vi "PhotonTrackedTarget_Pack.vi"(11 "TrackedTarget":T1={"Yaw"=0.0, "Pitch"=0.0, "Area"=0.0, "Skew"=0.0, "MinAreaRectCorners"=[], "BestCameraToTarget"={"TRANSLATION3D"={"X"=0.0, "Y"=0.0, "Z"=0.0}, "ROTATION3D"={"Q_quaternion"={"R"=1.0, "V"=[0.0, 0.0, 0.0]}}, "XF"=FALSE}, "FiducialId"=0, "AltCameraToTarget"={"TRANSLATION3D"={"X"=0.0, "Y"=0.0, "Z"=0.0}, "ROTATION3D"={"Q_quaternion"={"R"=1.0, "V"=[0.0, 0.0, 0.0]}}, "XF"=FALSE}, "PoseAmbiguity"=0.0, "DetectedCorners"=[], "ObjDetectId"=0, "ObjDetectConf"=0.0} {"AltCameraToTarget"."TRANSLATION3D"."Z" format="%14.3f"; "AltCameraToTarget"."TRANSLATION3D"."Y" format="%14.3f"; "AltCameraToTarget"."TRANSLATION3D"."X" format="%14.3f"; "BestCameraToTarget"."TRANSLATION3D"."Z" format="%14.3f"; "BestCameraToTarget"."TRANSLATION3D"."Y" format="%14.3f"; "BestCameraToTarget"."TRANSLATION3D"."X" format="%14.3f"}) -> (3 "RawData Out":u8[](array[numeric]))   [LabVIEW 2019, in "PhotonVisionLib.lvlib"]
doc: "Encode a TrackedTarget cluster into an array of bytes.\n\nInputs:\n - TrackedTarget -- TrackedTarget cluster.\n\nOutputs:\n - RawDataOut -- Byte array containing the encoded data."
uses:
  PhotonVisionLib.lvlib
  TypeDef/PhotonTrackedTargetType.ctl
  TypeDef/TargetCornerType.ctl
  <vilib>/Rock Robotics/WPI/ThirdParty/JAS_Junk/TrajLib/TypeDef/TRANSFORM3D.ctl
  <vilib>/Rock Robotics/WPI/ThirdParty/JAS_Junk/TrajLib/TypeDef/TRANSLATION3D.ctl
  <vilib>/Rock Robotics/WPI/ThirdParty/JAS_Junk/TrajLib/TypeDef/ROTATION3D.ctl
  <vilib>/Rock Robotics/WPI/ThirdParty/JAS_Junk/TrajLib/TypeDef/QUATERNION.ctl
  <vilib>/Rock Robotics/WPI/ThirdParty/JAS_Junk/TrajLib/VI/Transform3d_GetRotation3d.vi
  <vilib>/Rock Robotics/WPI/ThirdParty/JAS_Junk/TrajLib/VI/Transform3d_GetTranslation3d.vi
  <vilib>/Rock Robotics/WPI/ThirdParty/JAS_Junk/TrajLib/VI/Translation3d_ToTranslation2d.vi
  <vilib>/Rock Robotics/WPI/ThirdParty/JAS_Junk/TrajLib/VI/Rotation3d_ToRotation2d.vi
  <vilib>/Rock Robotics/WPI/ThirdParty/JAS_Junk/TrajLib/Transform2d_Create_TransRot.vi
  <vilib>/Rock Robotics/WPI/ThirdParty/JAS_Junk/TrajLib/VI/Transform3d_GetXYZ.vi
  <vilib>/Rock Robotics/WPI/ThirdParty/JAS_Junk/TrajLib/VI/Rotation3d_GetQuaterion.vi
  <vilib>/Rock Robotics/WPI/ThirdParty/JAS_Junk/TrajLib/VI/Quaternion_Get_All.vi
  Packet_encode_ByteI8.vi
  TargetCorner_GetAll.vi
  <vilib>/Rock Robotics/WPI/ThirdParty/JAS_Junk/TrajLib/Translation2d_Create.vi
  <vilib>/Rock Robotics/WPI/ThirdParty/JAS_Junk/TrajLib/Rotation2d_CreateAngle.vi
  <vilib>/Rock Robotics/WPI/ThirdParty/JAS_Junk/TrajLib/VI/Rotation3d_GetXYZ.vi
  <vilib>/Rock Robotics/WPI/ThirdParty/JAS_Junk/TrajLib/VI/Translation3d_GetXYZ.vi
  <vilib>/Rock Robotics/WPI/ThirdParty/JAS_Junk/TrajLib/Trajectory_Library.lvlib
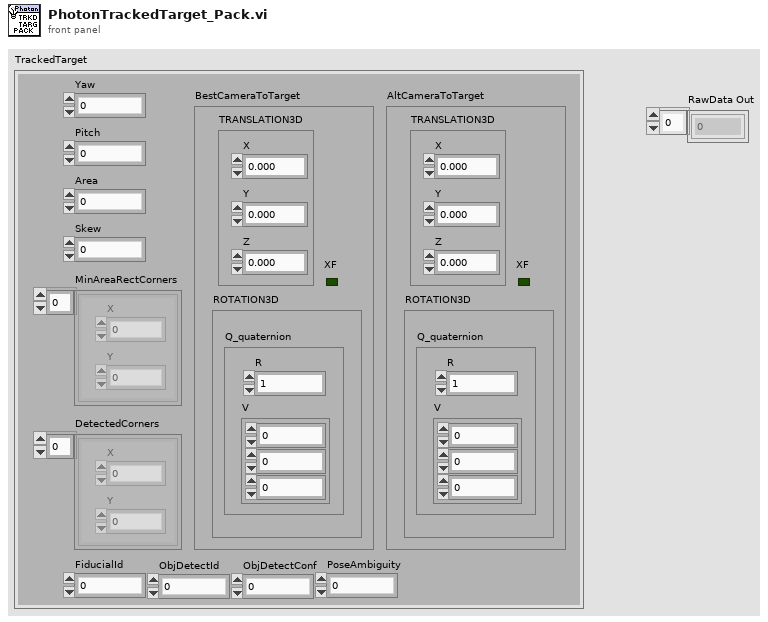
[diagram p1: front panel]
types:
  T1 = typedef "PhotonVisionLib.lvlib/PhotonTrackedTargetType.ctl" = cluster{"Yaw":dbl, "Pitch":dbl, "Area":dbl, "Skew":dbl, "MinAreaRectCorners":T2[], "BestCameraToTarget":T3, "FiducialId":i32, "AltCameraToTarget":T3, "PoseAmbiguity":dbl, "DetectedCorners":T2[], "ObjDetectId":i32, "ObjDetectConf":sgl}
  T2 = typedef "PhotonVisionLib.lvlib/TargetCornerType.ctl" = cluster{"X":dbl, "Y":dbl}
  T3 = typedef "Trajectory_Library.lvlib/TRANSFORM3D.ctl" = cluster{"TRANSLATION3D":T4, "ROTATION3D":T5, "XF":bool}
  T4 = typedef "Trajectory_Library.lvlib/TRANSLATION3D.ctl" = cluster{"X":dbl, "Y":dbl, "Z":dbl}
  T5 = typedef "Trajectory_Library.lvlib/ROTATION3D.ctl" = cluster{"Q_quaternion":T6}
  T6 = typedef "Trajectory_Library.lvlib/QUATERNION.ctl" = cluster{"R":dbl, "V":dbl[]}
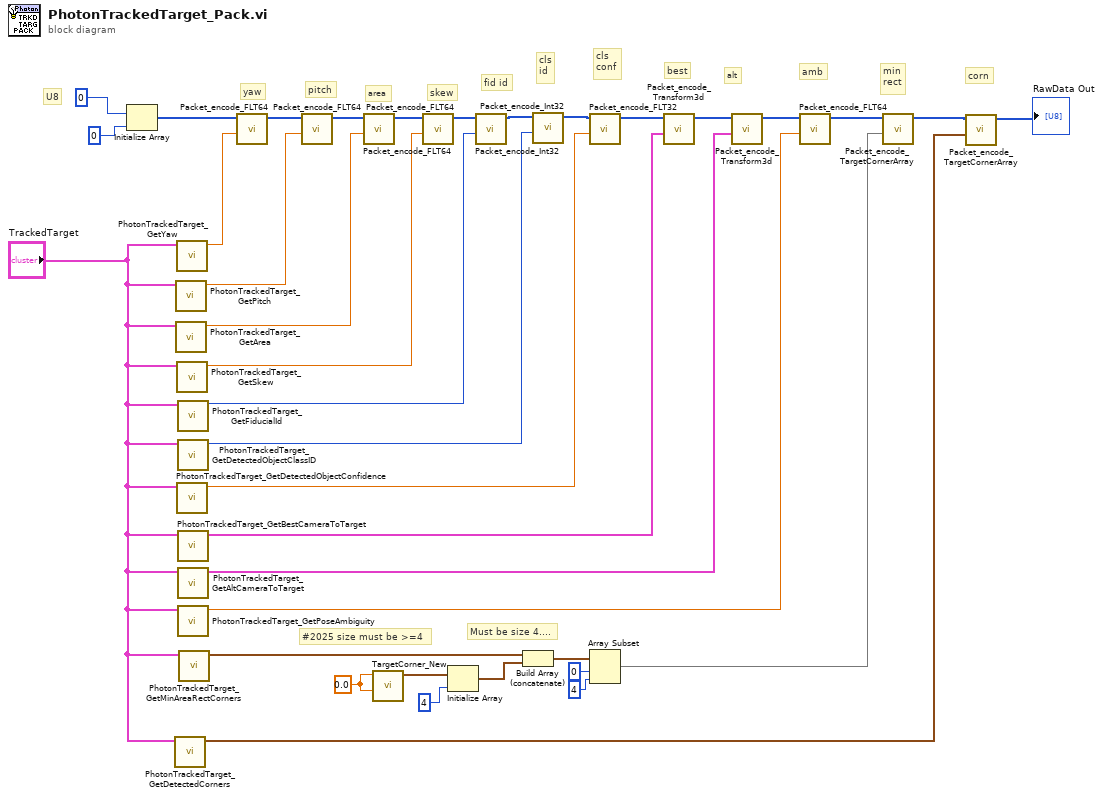
[diagram p0: block diagram]
diagram:
  w10 = 0.0 ("X")
  # "amb"
  # "Must be size 4...."
  # "#2025 size must be >=4"
  # "corn"
  # "min\nrect"
  # "alt"
  # "best"
  # "cls\nconf"
  # "cls\nid"
  # "fid id"
  # "skew"
  # "area"
  # "pitch"
  # "yaw"
  # "U8"
  n1 = Initialize Array(u8 0 ("element"), 0 ("dimension size")) -> (w34:u8[])
  n2 = call "PhotonTrackedTarget_GetDetectedCorners.vi"("TrackedTarget"="TrackedTarget") -> ("Detected Corners"=w14:T2[])  [unwired: 10 in]
  n3 = call "PhotonTrackedTarget_GetPitch.vi"("TrackedTarget"="TrackedTarget") -> ("Pitch"=w29:dbl)  [unwired: 10 in]
  n4 = call "PhotonTrackedTarget_GetArea.vi"("TrackedTarget"="TrackedTarget") -> ("Area"=w28:dbl)  [unwired: 10 in]
  n5 = call "PhotonTrackedTarget_GetYaw.vi"("TrackedTarget"="TrackedTarget") -> ("Yaw"=w30:dbl)  [unwired: 10 in]
  n6 = call "PhotonTrackedTarget_GetSkew.vi"("TrackedTarget"="TrackedTarget") -> ("Skew"=w27:dbl)  [unwired: 10 in]
  n7 = call "PhotonTrackedTarget_GetDetectedObjectConfidence.vi"("TrackedTarget"="TrackedTarget") -> ("DetectedObjectConfidence"=w16:sgl)  [unwired: 10 in]
  n8 = call "PhotonTrackedTarget_GetFiducialId.vi"("TrackedTarget"="TrackedTarget") -> ("Fiducial Id"=w25:i32)  [unwired: 10 in]
  n9 = call "PhotonTrackedTarget_GetDetectedObjectClassID.vi"("TrackedTarget"="TrackedTarget") -> ("DetectedObjectClassId"=w17:i32)  [unwired: 10 in]
  n10 = call "PhotonTrackedTarget_GetBestCameraToTarget.vi"("TrackedTarget"="TrackedTarget") -> ("BestCameraToTarget"=w23:T3)  [unwired: 9 in, 1 out]
  n11 = call "PhotonTrackedTarget_GetAltCameraToTarget.vi"("TrackedTarget"="TrackedTarget") -> ("AltCameraToTarget"=w22:T3)  [unwired: 9 in, 1 out]
  n12 = call "PhotonTrackedTarget_GetPoseAmbiguity.vi"("TrackedTarget"="TrackedTarget") -> ("Pose Ambiguity"=w1:dbl)  [unwired: 10 in]
  n13 = call "PhotonTrackedTarget_GetMinAreaRectCorners.vi"("TrackedTarget"="TrackedTarget") -> ("MinAreaRectCorners"=w5:T2[])  [unwired: 10 in]
  n14 = call "Packet_encode_FLT64.vi"("FLT64_Value"=w30, "RawData In"=w34) -> ("RawData Out"=w33:u8[])  [unwired: 9 in]
  n15 = call "Packet_encode_FLT64.vi"("FLT64_Value"=w29, "RawData In"=w33) -> ("RawData Out"=w32:u8[])  [unwired: 9 in]
  n16 = call "Packet_encode_FLT64.vi"("FLT64_Value"=w28, "RawData In"=w32) -> ("RawData Out"=w31:u8[])  [unwired: 9 in]
  n17 = call "TargetCorner_New.vi"("Y"=w10, "X"=w10) -> ("TargetCorner"=w12:T2)  [unwired: 9 in]
  n18 = call "Packet_encode_FLT64.vi"("FLT64_Value"=w27, "RawData In"=w31) -> ("RawData Out"=w26:u8[])  [unwired: 9 in]
  n19 = Initialize Array(w12, 4 ("dimension size")) -> (w9:T2[])
  n20 = call "Packet_encode_Int32.vi"("Int32_Value"=w25, "RawData In"=w26) -> ("RawData Out"=w21:u8[])  [unwired: 9 in]
  n21 = Build Array (concatenate)(w5, w9) -> (w8:T2[])
  n22 = call "Packet_encode_Int32.vi"("Int32_Value"=w17, "RawData In"=w21) -> ("RawData Out"=w20:u8[])  [unwired: 9 in]
  n23 = call "Packet_encode_FLT32.vi"("FLT32_Value"=w16, "RawData In"=w20) -> ("RawData Out"=w19:u8[])  [unwired: 9 in]
  n24 = Array Subset(array=w8, index=0, length=4) -> (w4:T2[])
  n25 = call "Packet_encode_Transform3d.vi"("Transform3d Value"=w23, "RawData In"=w19) -> ("RawData Out"=w24:u8[])  [unwired: 9 in]
  n26 = call "Packet_encode_Transform3d.vi"("Transform3d Value"=w22, "RawData In"=w24) -> ("RawData Out"=w3:u8[])  [unwired: 9 in]
  n27 = call "Packet_encode_FLT64.vi"("FLT64_Value"=w1, "RawData In"=w3) -> ("RawData Out"=w2:u8[])  [unwired: 9 in]
  n28 = call "Packet_encode_TargetCornerArray.vi"("TargetCornerArray"=w4, "RawData In"=w2) -> ("RawData Out"=w15:u8[])  [unwired: 9 in]
  n29 = call "Packet_encode_TargetCornerArray.vi"("TargetCornerArray"=w14, "RawData In"=w15) -> ("RawData Out"=→"RawData Out":u8[])  [unwired: 9 in]
